vi "set NR Mode for 8000A.vi"(8 "error in (no error)":errorcluster, 11 "NR in":refnum<class "NR.lvclass">) -> (0 "error out":errorcluster, 3 "NR out":refnum<class "NR.lvclass">)   [LabVIEW 2023, in "ANRITSU Call Box.lvlib" / "NR.lvclass"]
uses:
  NR.lvclass
  NR.lvclass/NR.ctl
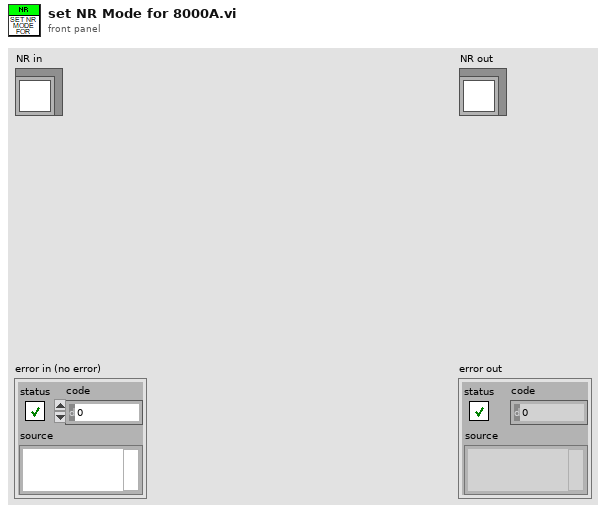
[diagram p1: front panel]
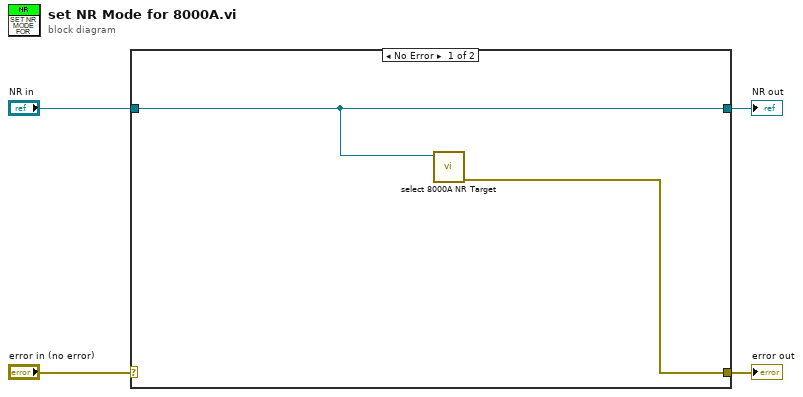
[diagram p0: block diagram]
diagram:
  n1 = case shown="No Error" "error in (no error)" {
    selector: "error in (no error)" -> [_ w8]
    tunnel: [w5 w8] -> w3
    tunnel: [w6 w7] -> w1
    tunnel: "NR in" -> [w6 w7]
    frame No Error {
      n2 = call "select 8000A NR Target.vi"("NR in"=w6) -> ("error out"=w5:errorcluster)  [unwired: 9 in, 1 out]
    }
    frame Error {
    }
  }
  "error out" <- w3
  "NR out" <- w1
